vi "VI Helpeks EULA.vi"   [LabVIEW 2014]
doc: "::: VI Helpeks :::\nCopyright (c) 2000-2026 Konstantin Shifershteyn. All rights reserved."
panel:
  # "VI Helpeks EULA"
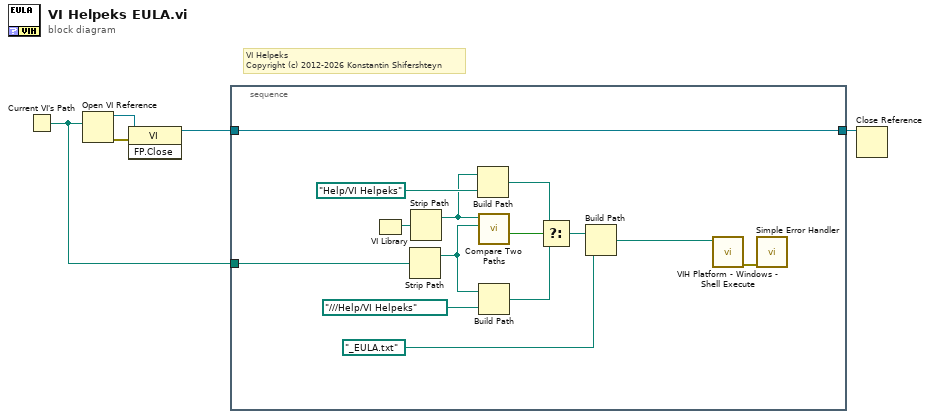
[diagram p0: block diagram]
diagram:
  # "VI Helpeks\nCopyright (c) 2012-2026 Konstantin Shifershteyn"
  n1 = Current VI's Path() -> (path=w1:path)
  n2 = Open VI Reference(vi path=w1) -> (vi reference=w4:refnum<vi>, error out=w5:errorcluster)  [unwired: 5 in]
  n3 = invoke class="VI" method="FP.Close"(reference=w4, error in=w5) -> (reference out=w3:refnum<vi>)  [unwired: 1 in, 2 out]
  n4 = stacked-sequence {
    tunnel: [w19] -> w2
    tunnel: w3 -> [w19]
    tunnel: w1 -> [w7]
    frame #0 {
      n5 = VI Library() -> (path=w8:path)
      n6 = Strip Path(path=w7) -> (stripped path=w15:path)  [unwired: 1 out]
      n7 = Strip Path(path=w8) -> (stripped path=w10:path)  [unwired: 1 out]
      n8 = Build Path(base path=w10, name or relative path=path "Help/VI Helpeks") -> (appended path=w12:path)
      n9 = call <vilib>:"Compare Two Paths.vi"("Path 2"=w15, "Path 1"=w10) -> ("Path 2 Relative to Path 1?"=w9:bool)  [unwired: 6 in, 3 out]
      n10 = Build Path(base path=w15, name or relative path=path "../../../Help/VI Helpeks") -> (appended path=w17:path)
      n11 = Select(t=w12, s=w9, f=w17) -> (s? t:f=w11:path)
      n12 = Build Path(base path=w11, name or relative path=path "_EULA.txt" ("append path")) -> (appended path=w6:path)
      n13 = call "VIH Platform - Windows - Shell Execute.vi"("exe/doc/dir path"=w6) -> ("error out"=w18:errorcluster)  [unwired: 10 in]
      n14 = call <vilib>:"Simple Error Handler.vi"("error in (no error)"=w18) -> ()  [unwired: 4 in, 5 out]
    }
  }
  n15 = Close Reference(reference=w2) -> ()  [unwired: 1 in, 1 out]
